vi "destroy.vi"(8 "error in (no error)":errorcluster, 11 "system.logging in":refnum<class "system.logging.lvclass">) -> (0 "error out":errorcluster)   [LabVIEW 2021, in "system.logging.lvclass"]
uses:
  system.logging.lvclass
  system.logging.lvclass/system.logging.ctl
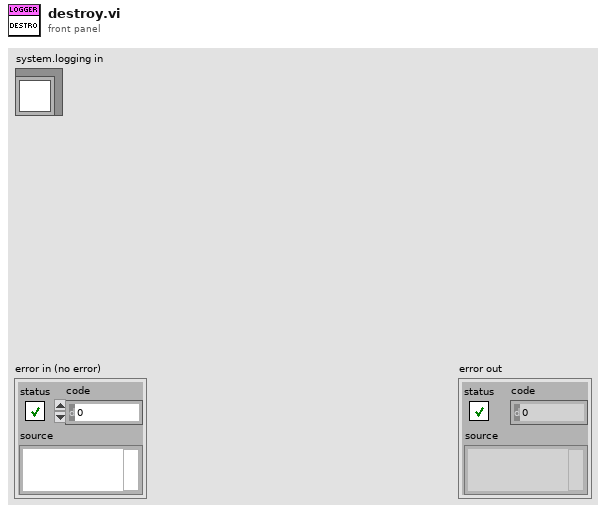
[diagram p1: front panel]
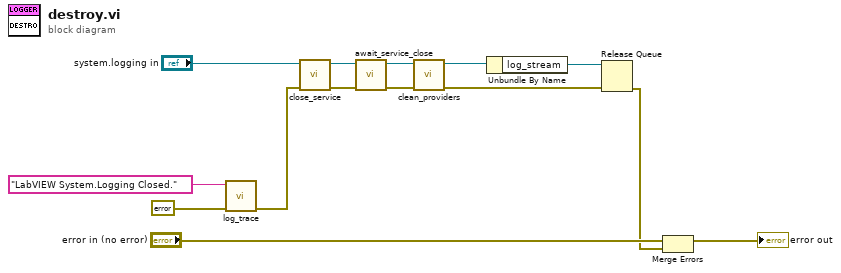
[diagram p0: block diagram]
diagram:
  n1 = call "log_trace.vi"("error in (no error)"=errorcluster {"status"=FALSE, "code"=0, "source"=""}, "message"="LabVIEW System.Logging Closed.") -> ("error out"=w2:errorcluster)  [unwired: 9 in]
  n2 = call "close_service.vi"("error in (no error)"=w2, "system.logging (in)"="system.logging in") -> ("error out"=w10:errorcluster, "system.logging (out)"=w11:refnum<class "system.logging.lvclass">)  [unwired: 8 in]
  n3 = call "await_service_close.vi"("error in (no error)"=w10, "system.logging in"=w11) -> ("error out"=w8:errorcluster, "system.logging out"=w9:refnum<class "system.logging.lvclass">)  [unwired: 8 in]
  n4 = call "clean_providers.vi"("error in (no error)"=w8, "system.logging in"=w9) -> ("error out"=w5:errorcluster, "system.logging out"=w7:refnum<class "system.logging.lvclass">)  [unwired: 8 in]
  n5 = Unbundle By Name(w7) -> ("log_stream"=w6:refnum<queue>)
  n6 = Release Queue(queue=w6, error in (no error)=w5) -> (error out=w4:errorcluster)  [unwired: 1 in, 2 out]
  n7 = Merge Errors("error in (no error)", w4) -> (→"error out":errorcluster)
